vi "[ce] CalcExpress - Variables Writer ID.vi"(6 "set (F)":bool, 8 "error in":errorcluster, 10 "writer ID in":u32, 11 "CE InstanceRef":T1) -> (0 "error out":errorcluster, 2 "writer ID out":u32, 3 "dup CE InstanceRef":T1)   [LabVIEW 2021]
doc: "Use this VI to preset the <b>writer ID</b> used by the given CE Instance for writing to variables during execution. The <b>writer ID</b> can also be modified using the <b>vwrid(wrid)</b> function in an expression/script. Refer to the VI help for more details.\n\n<b>writer ID in</b> control specifies the value to preset.\n\n<b>writer ID out</b> indicator returns the actual value.\n\n<b>set (F)</b> control defines the action to perform. If FALSE (default), the VI returns the actual writer ID; otherwise, it sets a new value from the <b>writer ID in</b> control.\n\n::: CalcExpress Toolkit :::\nCopyright (c) 2000-2026 Konstantin Shifershteyn. All rights reserved."
uses:
  cetypes.llb/CalcExpress Instance RefNum.ctl
  cersrc/celveng32.dll
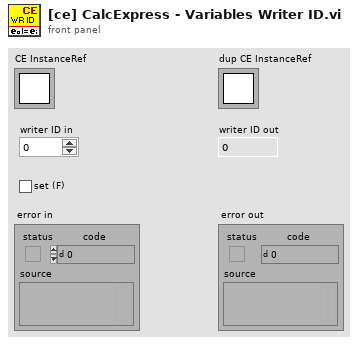
[diagram p1: front panel]
types:
  T1 = typedef "CalcExpress Instance RefNum.ctl" = refnum<k1>
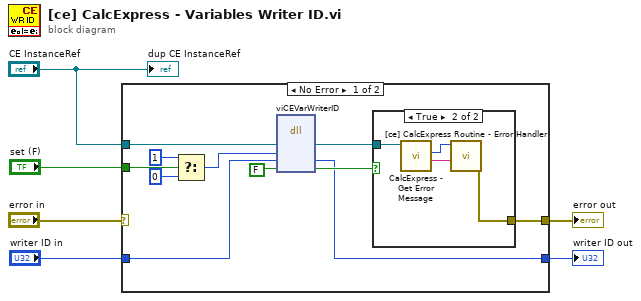
[diagram p0: block diagram]
diagram:
  n1 = case shown="No Error" "error in" {
    selector: "error in" -> [_ w23]
    tunnel: [w16 w23] -> w6
    tunnel: "CE InstanceRef" -> [w15 _]
    tunnel: "set (F)" -> [w10 _]
    tunnel: "writer ID in" -> [w8 w22]
    tunnel: [w7 w22] -> w1
    frame No Error {
      n2 = Select(t=1, s=w10, f=0) -> (s? t:f=w9:i32)
      n3 = dll-call lib="C:/LV Projects/CalcExpress 40 LV2021/vi.lib/addons/CalcExpress/cersrc/celveng*.dll" fn="viCEVarWriterID" ("viCEDiagExp")("iRef"=w15, "cmd"=w9, "writerID"=w8, FALSE) -> ("iRef"=w17:T1, "writerID"=w7:u32, w13:bool)  [unwired: 5 in, 2 out]
      n4 = case shown="True" w13 {
        tunnel: [_ w21] -> w16
        tunnel: w17 -> [_ w19]
        frame False {
        }
        frame True {
          n5 = call "CalcExpress - Get Error Message.vi"("CE InstanceRef"=w19) -> ("error description"=w20:string, "error code"=w18:i32)  [unwired: 5 in, 2 out]
          n6 = call "[ce] CalcExpress Routine - Error Handler.vi"("error msg"=w20, "error code"=w18) -> ("error out"=w21:errorcluster)  [unwired: 7 in]
        }
      }
    }
    frame Error {
    }
  }
  "error out" <- w6
  "writer ID out" <- w1
  "dup CE InstanceRef" <- "CE InstanceRef"
